vi "fake tool schema shapes.vi"(7 "mode":enum16{"slow", "fast"}(ring), 8 "matrix":i32[][](array[numeric]), 9 "variants":variant[](array[variant]), 10 "settings":T1, 11 "timestamp":timestamp) -> (0 "mode out":enum16{"slow", "fast"}(ring), 1 "matrix out":i32[][](array[numeric]), 2 "settings out":T1, 3 "time out":timestamp, 4 "variant count":i32)   [LabVIEW 2020, in "MCP Server tests.lvlib"]
doc: "Fake tool to test the JSON schema of types beyond plain numbers, strings and Booleans, and the conversion of their arguments in tools/call: a timestamp, a cluster that contains a cluster with a timestamp and an array of clusters, an array of variants (no JSON type), a 2D array of I32 and a U16 enum. Each input is returned unchanged on an output, so a tools/call answer shows how the argument arrived."
uses:
  MCP Server tests.lvlib
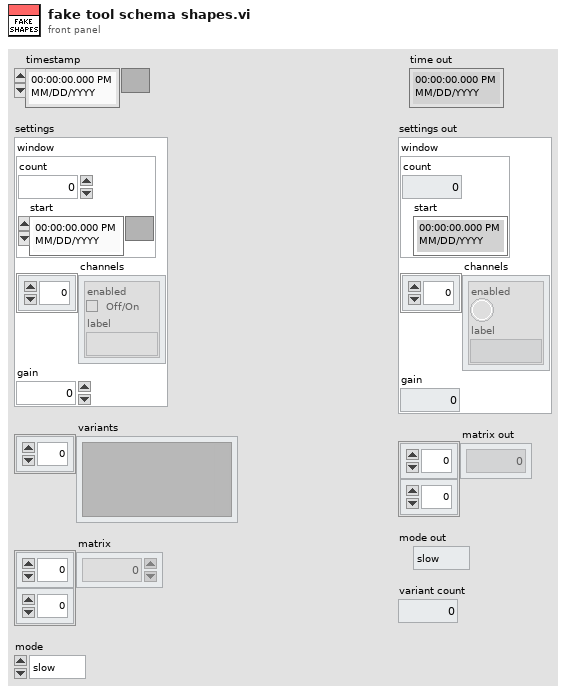
[diagram p1: front panel]
types:
  T1 = cluster{"window":cluster{"count":i32, "start":timestamp}, "channels":cluster{"enabled":bool, "label":string}[], "gain":dbl}
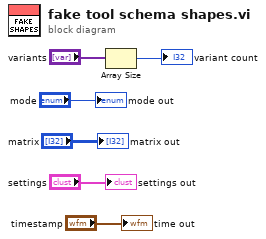
[diagram p0: block diagram]
diagram:
  n1 = Array Size(array="variants") -> (size(s)=→"variant count":i32)
  "time out" <- "timestamp"
  "settings out" <- "settings"
  "matrix out" <- "matrix"
  "mode out" <- "mode"
